vi "SetPath.vi"(8 "error in (no error)":errorcluster, 10 "path to MRU item":path, 11 "MRU in":refnum<class "MRU.lvclass">) -> (0 "error out":errorcluster, 3 "MRU out":refnum<class "MRU.lvclass">)   [LabVIEW 2023, in "GettingStartedWindow.lvlib" / "MRU.lvclass"]
uses:
  <resource>/modes/FRC/Classes/MRU/MRU.lvclass
  <resource>/modes/FRC/Classes/MRU/MRU.lvclass/MRU.ctl
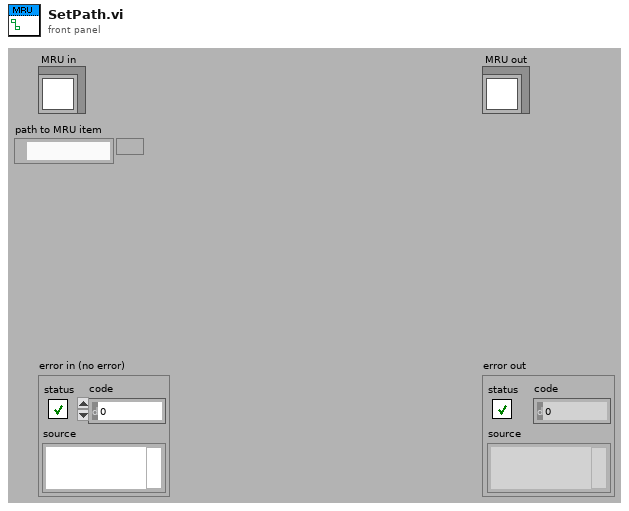
[diagram p1: front panel]
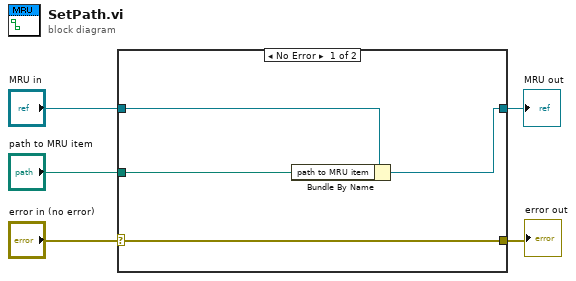
[diagram p0: block diagram]
diagram:
  n1 = case shown="No Error" "error in (no error)" {
    selector: "error in (no error)" -> [w9 w11]
    tunnel: [w9 w11] -> w4
    tunnel: [w6 w10] -> w2
    tunnel: "MRU in" -> [w8 w10]
    tunnel: "path to MRU item" -> [w7 _]
    frame No Error {
      n2 = Bundle By Name(cluster=w8, "path to MRU item"=w7) -> (w6:refnum<class "MRU.lvclass">)
    }
    frame Error {
    }
  }
  "error out" <- w4
  "MRU out" <- w2
